vi "GetCurrentThreadId Wrapper Template.vi"(11 "error in":errorcluster) -> (4 "thread ID":u32, 15 "error out":errorcluster)   [LabVIEW 2020]
doc: "Returns the identifier of the calling thread through kernel32.dll GetCurrentThreadId (stdcall, called in LabVIEW's UI thread, so it is the UI thread's identifier - the thread whose key state user32 SetKeyboardState.vi writes). When error in carries an error the DLL is not called. Generated by scripts\\Build Win32 Wrappers.vi - do not edit by hand, rebuild it."
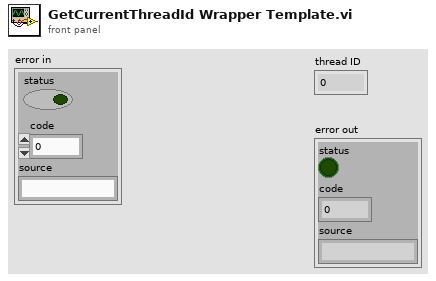
[diagram p1: front panel]
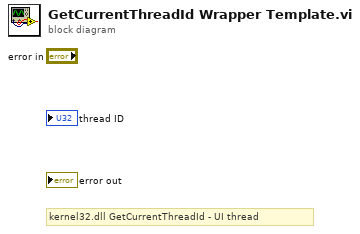
[diagram p0: block diagram]
diagram:
  # "kernel32.dll GetCurrentThreadId - UI thread"
